vi "Import Scalars - by label.vi"(8 "error in":errorcluster, 10 "bitfile scalars in":T1[](array[typedef]), 11 "FPGA addon refnum in":T4=18446744073709551615 format="%.0x") -> (0 "error out":errorcluster, 2 "imported bitfile scalars out":T2[](array[typedef]), 3 "FPGA addon refnum out":T4=18446744073709551615 format="%.0x")   [LabVIEW 2020, in "Scripting API.lvlib"]
doc: "Imports the specified control and indicator registers. The function operates only on scalar objects. For each control or indicator, a channel will be created within the target FPGA addon, under their respective section (Scalar Inputs or Scalar Outputs). By default (i.e. if the \"SysDef Name\" field for a given scalar is empty) the channel names will correspond to the control and indicator labels within the bitfile. The input Bitfile and SysDef names must be unique, otherwise this VI will throw an error.\n\nOnce the import is complete, this function returns an array containing bitfile (control and indicator) registers data, and whether they were imported or not."
uses:
  Scripting API.lvlib
  <vilib>/NI VeriStand/Custom Device API/Custom Device Item Ref.ctl
  TypeDefs/Output Scalar Data.ctl
  Addon/Addon Shared/Types/FPGA Addon Data Type.ctl
  TypeDefs/Input Scalar Data.ctl
  Addon/Addon Shared/Types/FG Action.ctl
  Addon/Addon Shared/SubVIs/Constants.vi
  <vilib>/NI VeriStand/Custom Device API/NI VeriStand - Get Item Property.vi
  <vilib>/NI VeriStand/Custom Device API/Get Item Property (Path).vi
  <vilib>/NI VeriStand/Custom Device API/Get Item Property (String).vi
  <vilib>/NI VeriStand/Custom Device API/Get Item Property (Boolean).vi
  <vilib>/NI VeriStand/Custom Device API/NI VeriStand - Set Item Property.vi
  <vilib>/NI VeriStand/Custom Device API/Set Item Property (Path).vi
  <vilib>/NI VeriStand/Custom Device API/Set Item Property (String).vi
  <vilib>/NI VeriStand/Custom Device API/Set Item Property (Boolean).vi
  Addon/Addon Shared/FPGA Addon Shared.lvlib
  <vilib>/NI VeriStand/Custom Device API/Custom Device API.lvlib
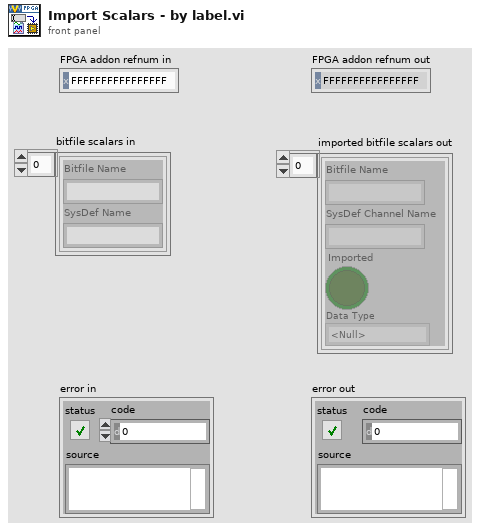
[diagram p1: front panel]
types:
  T1 = typedef "Scripting API.lvlib/Input Scalar Data.ctl" = cluster{"Bitfile Name":string, "SysDef Name":string}
  T2 = typedef "Scripting API.lvlib/Output Scalar Data.ctl" = cluster{"Bitfile Name":string, "SysDef Channel Name":string, "Imported":bool, "Data Type":T3}
  T3 = typedef "FPGA Addon Shared.lvlib/FPGA Addon Data Type.ctl" = enum8{"<Null>", "I8", "I16", "I32", "I64", "U8", "U16", "U32", "U64", "SGL", "Boolean", "Analog PWM In Settings", "Analog PWM In", "Digital PWM In Settings", "Digital PWM In", "Digital PWM Out", "Sine Out", "FXP", "FXP+/-24.5", "FXP+/-16.5", "FXP+/-32.8", "FXP+/-64.32", "FXP+/-16.7", "FXP+/-20.5", "FXP+/-27.5", "FXP+/-32.16", "FXP+16.3", "FXP+18.3", "Digital Static In", "Digital Static Out", "Digital Static In Settings", "Digital WSS Out", "Quad Encoder Settings", "Quad Encoder In", "Group"}
  T4 = typedef "Custom Device API.lvlib/Custom Device Item Ref.ctl" = u64
  T5 = typedef "FPGA Addon Shared.lvlib/FG Action.ctl" = enum8{"GET", "SET"}
  T6 = typedef "FPGA Addon Shared.lvlib/FPGA Settings.ctl" = cluster{"Bitfile path":path, "RIO Device Address":string, "Group":bool}
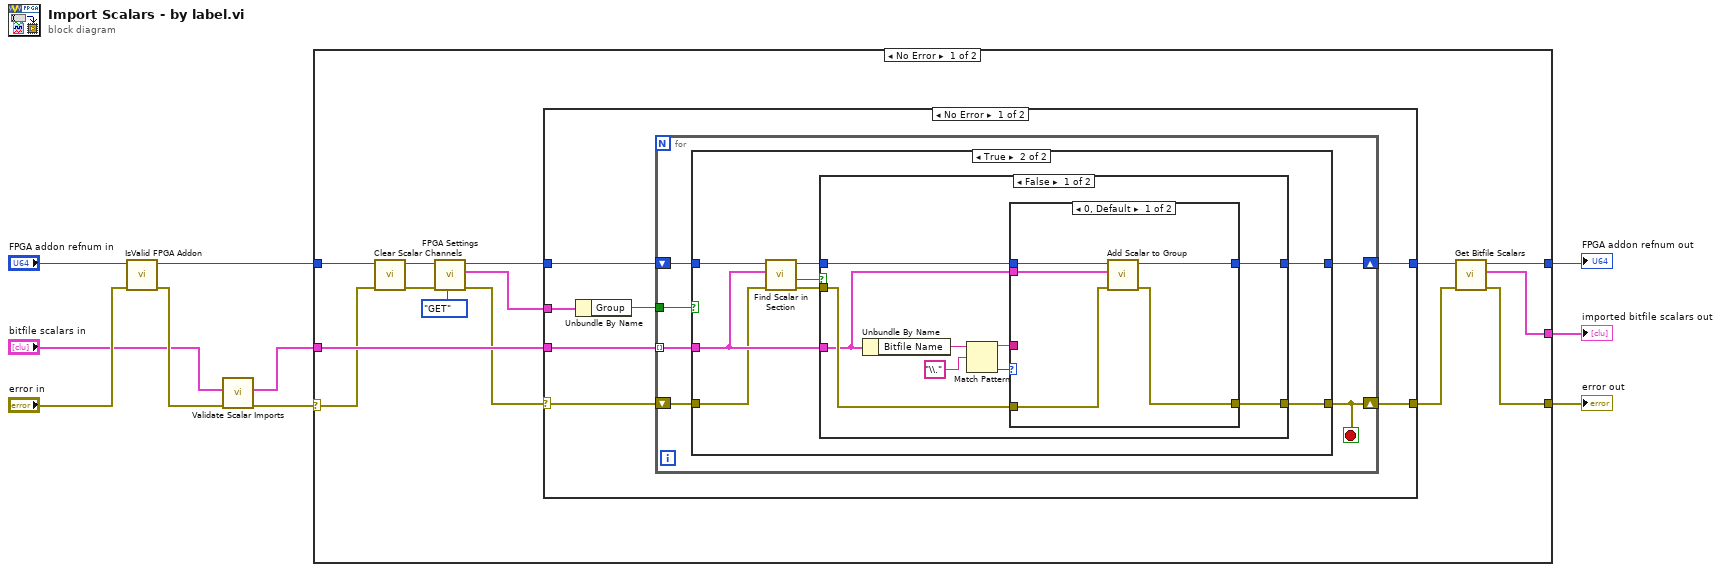
[diagram p0: block diagram]
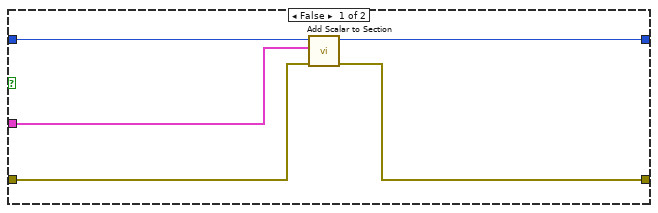
[diagram p2: hidden frame]
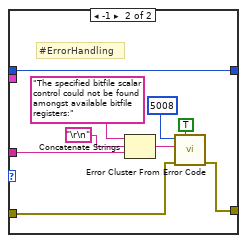
[diagram p3: hidden frame]
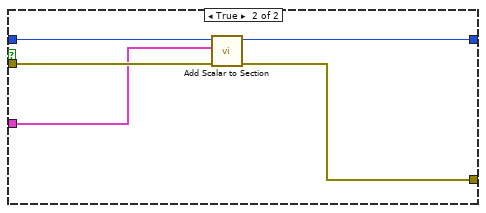
[diagram p4: hidden frame]
diagram:
  n1 = call "IsValid FPGA Addon.vi"("error in"="error in", "FPGA Addon refnum in"="FPGA addon refnum in") -> ("error out"=w4:errorcluster, "FPGA Addon refnum out"=w8:T4)  [unwired: 8 in]
  n2 = call "Validate Scalar Imports.vi"("error in (no error)"=w4, "bitfile scalars in"="bitfile scalars in") -> ("error out"=w3:errorcluster, "bitfile scalars out"=w5:T1[])  [unwired: 8 in]
  n3 = case shown="No Error" w3 {
    selector: w3 -> [w13 w81]
    tunnel: w8 -> [w14 w82]
    tunnel: w5 -> [w24 _]
    tunnel: [w16 w81] -> w6
    tunnel: [w18 w82] -> w7
    tunnel: [w15 _] -> w2
    frame No Error {
      n4 = call "Clear Scalar Channels.vi"("error in"=w13, "FPGA Addon refnum in"=w14) -> ("error out"=w11:errorcluster, "FPGA Addon refnum out"=w12:T4)  [unwired: 8 in]
      n5 = call "FPGA Settings.vi"("Action"=FG_Action."GET", "error in (no error)"=w11, "Item Ref"=w12) -> ("error out"=w20:errorcluster, "FPGA Settings"=w22:T6, "Item Ref out"=w21:T4)  [unwired: 6 in]
      n6 = case shown="No Error" w20 {
        selector: w20 -> [w27 w79]
        tunnel: w24 -> [w31 _]
        tunnel: w22 -> [w30 _]
        tunnel: w21 -> [w25 w80]
        tunnel: [w28 w79] -> w17
        tunnel: [w26 w80] -> w19
        frame No Error {
          n7 = Unbundle By Name(w30) -> ("Group"=w29:bool)
          n8 = for {
            tunnel: w31 -> [w36] mode=indexing
            shift-right: [w37] -> w26
            shift-left: w25 -> [w35]
            tunnel: w29 -> [w33]
            shift-right: [w32] -> w28
            shift-left: w27 -> [w34]
            stop <- w32 stop-if-true
            n9 = case shown="True" w33 {
              tunnel: w36 -> [w41 w47]
              tunnel: w35 -> [w42 w48]
              tunnel: w34 -> [w40 w46]
              tunnel: [w39 w50] -> w37
              tunnel: [w38 w49] -> w32
              frame False {
                n10 = call "Add Scalar to Section.vi"("error in"=w40, "Scalar Data"=w41, "Item Ref in"=w42) -> ("error out"=w38:errorcluster, "Item Ref out"=w39:T4)  [unwired: 7 in]
              }
              frame True {
                n11 = call "Find Scalar in Section.vi"("error in"=w46, "Scalar Data"=w47, "FPGA Addon refnum in"=w48) -> ("error out"=w43:errorcluster, "Found ?"=w45:bool, "FPGA Addon refnum out"=w44:T4)  [unwired: 5 in, 1 out]
                n12 = case shown="False" w45 {
                  tunnel: [w59 w76] -> w50
                  tunnel: [w58 w74] -> w49
                  tunnel: w47 -> [w53 w75]
                  tunnel: w44 -> [w57 w78]
                  tunnel: w43 -> [w56 w77]
                  frame False {
                    n13 = Unbundle By Name(w53) -> ("Bitfile Name"=w55:string)
                    n14 = Match Pattern(string=w55, regular expression="\\.") -> (before substring=w51:string, offset past match=w52:i32)  [unwired: 1 in, 2 out]
                    n15 = case shown="0, Default" w52 {
                      tunnel: [w64 w73] -> w59
                      tunnel: [w63 w65] -> w58
                      tunnel: w57 -> [w62 w73]
                      tunnel: w56 -> [w61 w66]
                      tunnel: w53 -> [w60 _]
                      tunnel: w51 -> [_ w67]
                      frame 0, Default {
                        n16 = call "Add Scalar to Group.vi"("error in"=w61, "Scalar Data"=w60, "FPGA Addon refnum in"=w62) -> ("error out"=w63:errorcluster, "FPGA Addon refnum out"=w64:T4)  [unwired: 6 in, 1 out]
                      }
                      frame -1 {
                        # "#ErrorHandling"
                        n17 = Concatenate Strings("The specified bitfile scalar control could not be found amongst available bitfile registers:" ("error message (\"\")"), "\r\n", w67) -> (w72:string)
                        n18 = call <vilib>:"Error Cluster From Error Code.vi"("show call chain? (False)"=TRUE, "error in (no error)"=w66, "error message (\"\")"=w72, "error code (0)"=5008) -> ("error out"=w65:errorcluster)  [unwired: 5 in]
                      }
                    }
                  }
                  frame True {
                    n19 = call "Add Scalar to Section.vi"("error in"=w77, "Scalar Data"=w75, "Item Ref in"=w78) -> ("error out"=w74:errorcluster, "Item Ref out"=w76:T4)  [unwired: 7 in]
                  }
                }
              }
            }
          }
        }
        frame Error {
        }
      }
      n20 = call "Get Bitfile Scalars.vi"("error in"=w17, "FPGA addon refnum in"=w19) -> ("error out"=w16:errorcluster, "bitfile scalars out"=w15:T2[], "FPGA addon refnum out"=w18:T4)  [unwired: 7 in]
    }
    frame Error {
    }
  }
  "error out" <- w6
  "FPGA addon refnum out" <- w7
  "imported bitfile scalars out" <- w2
